vi "DuplicateClientNames.vi"() -> (2 "one select refnum":refnum<vi>, 3 "all select refnum":refnum<vi>)   [LabVIEW 2021]
panel:
  in  "Multicolumn Listbox 2":i32(listbox)
  in  "Multicolumn Listbox":i32(listbox)
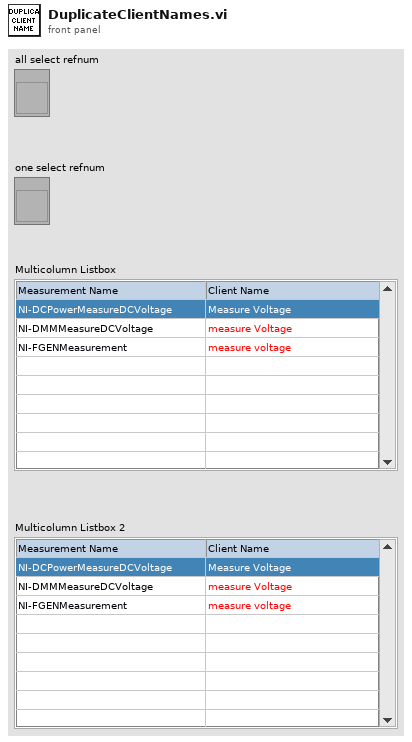
[diagram p1: front panel]
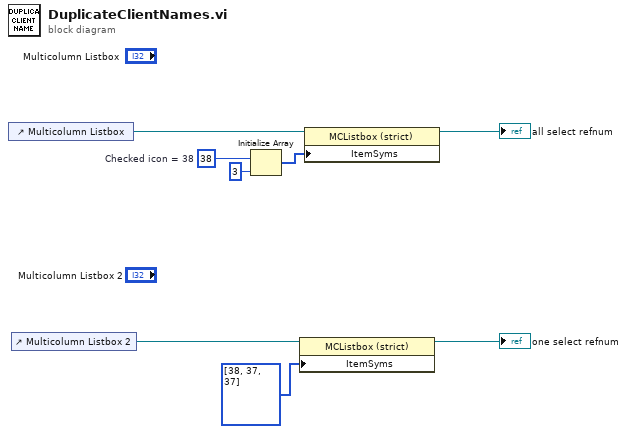
[diagram p0: block diagram]
diagram:
  w6 = 38  # Checked icon = 38
  n1 = control-ref of="Multicolumn Listbox"() -> (w8:refnum<vi>)
  n2 = control-ref of="Multicolumn Listbox 2"() -> (w3:refnum<vi>)
  n3 = Initialize Array(w6, 3 ("dimension size")) -> (w4:i32[])
  n4 = property class="MCListbox (strict)"(reference=w3, "ItemSyms"=i32[] [38, 37, 37]) -> (reference out=→"one select refnum":refnum<vi>)  [unwired: 1 in, 1 out]
  n5 = property class="MCListbox (strict)"(reference=w8, "ItemSyms"=w4) -> (reference out=→"all select refnum":refnum<vi>)  [unwired: 1 in, 1 out]
